vi "Create Channel.vi"(8 "error in (no error)":errorcluster, 10 "DIO_CFG":refnum<class "DIO-Configuration.lvclass">, 11 "UI Template in":refnum<class "DIO_Panel.lvclass">) -> (0 "error out":errorcluster, 3 "UI Template out":refnum<class "DIO_Panel.lvclass">)   [LabVIEW 2021, in "Simulator-Channel.lvlib" / "DIO_Panel.lvlib" / "DIO_Panel.lvclass"]
uses:
  DIO_Panel.lvclass
  Dependencies/DIO-Channel.lvlibp/Channels/DIO-Channel/DIO-Configuration_class/DIO-Configuration.lvclass
  C:/Users/averna/Documents/LV Gym DEMO/Factory Pattern/Channels/Dependencies/Channel.lvlibp/Channel/Configuration_class/Configuration.lvclass
  DIO_Panel.lvclass/DIO_Panel.ctl
  tdef/info.ctl
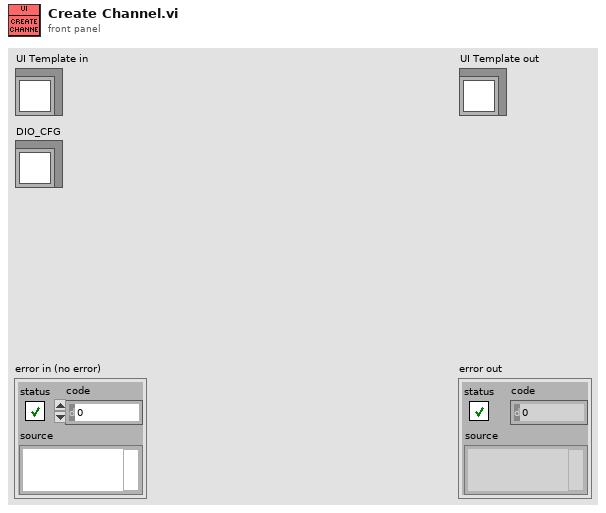
[diagram p1: front panel]
types:
  T1 = typedef "Simulator-Channel.lvlib/DIO_Panel.lvlib/DIO_Panel.lvclass/info.ctl" = cluster{"Name":string, "Boolean":bool}
  T2 = typedef "DIO-Channel.lvlibp/DIO-Configuration.lvclass/Direction.ctl" = enum16{"Input", "Output"}
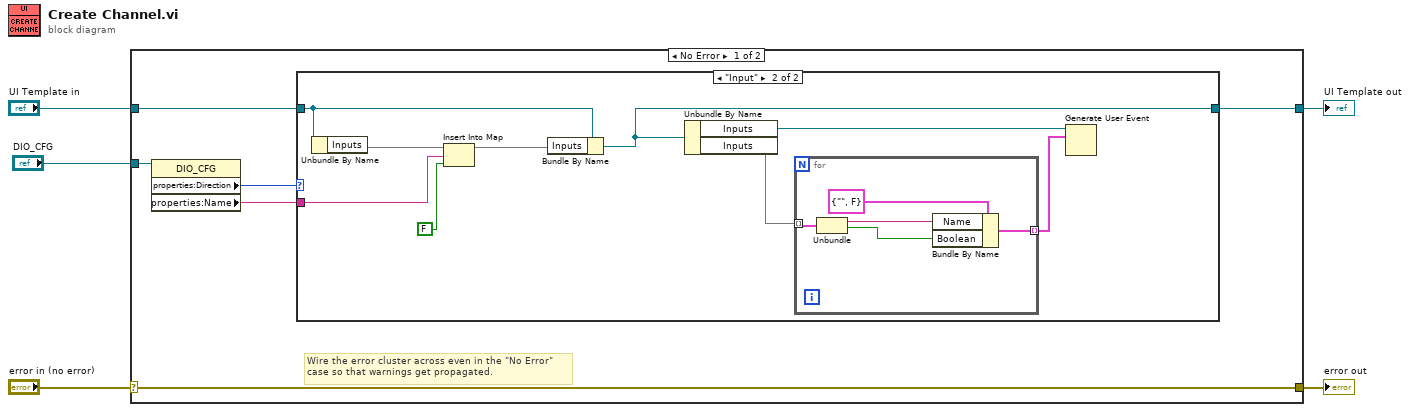
[diagram p0: block diagram]
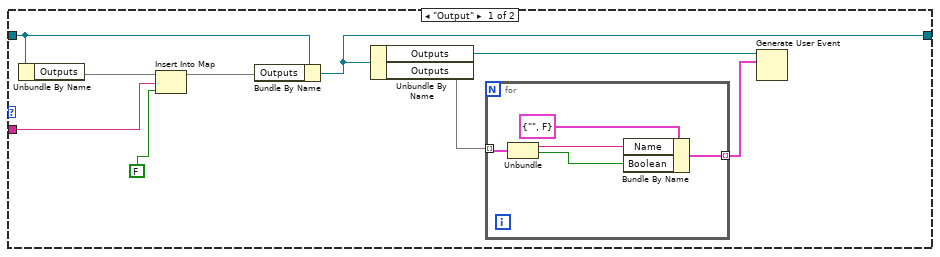
[diagram p2: hidden frame]
diagram:
  n1 = case shown="No Error" "error in (no error)" {
    selector: "error in (no error)" -> [w11 w41]
    tunnel: [w11 w41] -> w4
    tunnel: [w9 w40] -> w2
    tunnel: "UI Template in" -> [w8 w40]
    tunnel: "DIO_CFG" -> [w10 _]
    frame No Error {
      # "Wire the error cluster across even in the \"No Error\"\ncase so that warnings get propagated."
      n2 = property class="DIO_CFG"(reference=w10) -> ("properties:Direction"=w7:T2, "properties:Name"=w6:string)  [unwired: 1 in, 2 out]
      n3 = case shown="\"Input\"" w7 {
        tunnel: [w12 w26] -> w9
        tunnel: w8 -> [w20 w34]
        tunnel: w6 -> [w17 w31]
        frame "Output" {
          n4 = Unbundle By Name(w20) -> ("Outputs"=w19:map{string, bool})
          n5 = Insert Into Map(map in=w19, key=w17, value=FALSE) -> (map out=w18:map{string, bool})  [unwired: 2 out]
          n6 = Bundle By Name(cluster=w20, "Outputs"=w18) -> (w12:refnum<class "DIO_Panel.lvclass">)
          n7 = Unbundle By Name(w12) -> ("Outputs"=w14:refnum<user-event>, "Outputs"=w15:map{string, bool})
          n8 = for {
            tunnel: w15 -> [w25] mode=indexing
            tunnel: [w21] -> w13 mode=indexing
            n9 = Unbundle(w25) -> (w23:string, "Boolean"=w22:bool)
            n10 = Bundle By Name(cluster=T1 {"Name"="", "Boolean"=FALSE} ("Info"), "Name"=w23, "Boolean"=w22) -> (w21:T1)
          }
          n11 = Generate User Event(user event=w14, event data cluster=w13) -> ()  [unwired: 2 in, 2 out]
        }
        frame "Input" {
          n12 = Unbundle By Name(w34) -> ("Inputs"=w33:map{string, bool})
          n13 = Insert Into Map(map in=w33, key=w31, value=FALSE) -> (map out=w32:map{string, bool})  [unwired: 2 out]
          n14 = Bundle By Name(cluster=w34, "Inputs"=w32) -> (w26:refnum<class "DIO_Panel.lvclass">)
          n15 = Unbundle By Name(w26) -> ("Inputs"=w28:refnum<user-event>, "Inputs"=w29:map{string, bool})
          n16 = for {
            tunnel: w29 -> [w39] mode=indexing
            tunnel: [w35] -> w27 mode=indexing
            n17 = Unbundle(w39) -> (w37:string, "Boolean"=w36:bool)
            n18 = Bundle By Name(cluster=T1 {"Name"="", "Boolean"=FALSE} ("Info"), "Name"=w37, "Boolean"=w36) -> (w35:T1)
          }
          n19 = Generate User Event(user event=w28, event data cluster=w27) -> ()  [unwired: 2 in, 2 out]
        }
      }
    }
    frame Error {
    }
  }
  "error out" <- w4
  "UI Template out" <- w2
